vi "REST_Expect.vi"(7 "expected":i32=200, 8 "error in (no error)":errorcluster, 9 "response":string, 10 "what":string, 11 "status":i32) -> (0 "error out":errorcluster, 3 "ok":bool)   [LabVIEW 2021, in "CANsub_Common.lvlib"]
doc: "Checks the HTTP status of a CANsub REST call. If it is not the expected value, sets error 5000 with the call name, the status and the response. An incoming error is kept first."
uses:
  CANsub_Common.lvlib
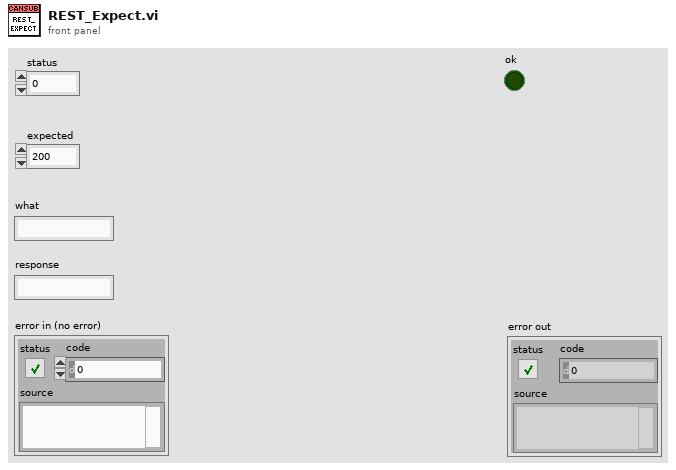
[diagram p1: front panel]
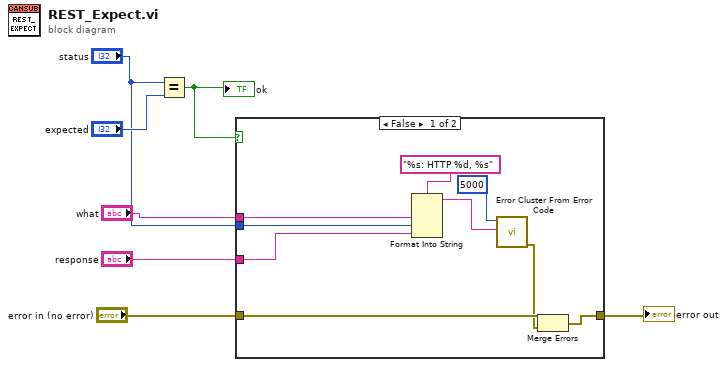
[diagram p0: block diagram]
diagram:
  n1 = Equal?(x="status", y="expected") -> (x = y?=w6:bool)
  "ok" <- w6
  n2 = case shown="False" w6 {
    tunnel: "error in (no error)" -> [w13 w17]
    tunnel: [w11 w17] -> w4
    tunnel: "status" -> [w10 _]
    tunnel: "what" -> [w9 _]
    tunnel: "response" -> [w8 _]
    frame False {
      n3 = Format Into String(format string="%s: HTTP %d, %s", w9, w10, w8) -> (resulting string=w15:string)  [unwired: 2 in, 1 out]
      n4 = call <vilib>:"Error Cluster From Error Code.vi"("error message (\"\")"=w15, "error code (0)"=5000) -> ("error out"=w12:errorcluster)  [unwired: 7 in]
      n5 = Merge Errors(w13, w12) -> (w11:errorcluster)
    }
    frame True {
    }
  }
  "error out" <- w4
